vi "Make HTTP Request v4.vi"(5 "Request Options":T1={"request headers"=[], "request parameters"=[], "request body"="", "region handling"=enum."use region everywhere", "URL formatting"=enum."region."}, 7 "HTTP-Verb":string(combo)="GET", 8 "error in":errorcluster, 9 "URL Suffix":string, 10 "URL Prefix":string, 11 "AWS Core in":refnum<class "HTTP Request.lvclass">) -> (0 "error out":errorcluster, 1 "response body":string, 2 "response headers":string, 3 "AWS Core out":refnum<class "HTTP Request.lvclass">, 4 "Call Result":string)   [LabVIEW 2015, in "NI_AWS_Core.lvlib" / "HTTP Request.lvclass"]
uses:
  HTTP Request.lvclass
  Request Options.ctl
  Name Value Pair.ctl
  Region handling.ctl
  URL formatting.ctl
  HTTP Request.lvclass/HTTP Request.ctl
  Read Credentials.vi
  Read Service.vi
  Read Verify Server.vi
  <vilib>/httpClient/LabVIEWHTTPClient.lvlib
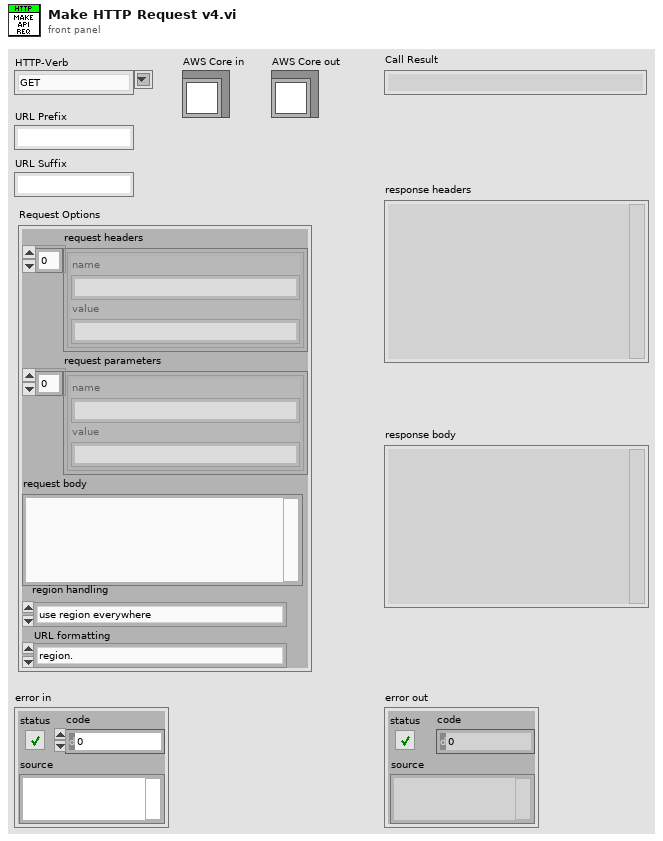
[diagram p1: front panel]
types:
  T1 = typedef "NI_AWS_Core.lvlib/HTTP Request.lvclass/Request Options.ctl" = cluster{"request headers":T2[], "request parameters":T2[], "request body":string, "region handling":T3, "URL formatting":T4}
  T2 = typedef "NI_AWS_Core.lvlib/HTTP Request.lvclass/Name Value Pair.ctl" = cluster{"name":string, "value":string}
  T3 = typedef "NI_AWS_Core.lvlib/HTTP Request.lvclass/Region handling.ctl" = enum16{"use region everywhere", "use region (authentication only)", "use region (URL only)", "ignore region everwhere"}
  T4 = typedef "NI_AWS_Core.lvlib/HTTP Request.lvclass/URL formatting.ctl" = enum16{"region-", "region."}
  T5 = typedef "AWS Core.lvlib/AWS Credentials.ctl" = cluster{"Access Key":string, "Secret Key":string}
  T6 = typedef "NI_AWS_Core.lvlib/HTTP Request.lvclass/Region.ctl" = enum16{"us-east-1", "us-east-2", "us-west-1", "us-west-2", "ap-northeast-1", "ap-northeast-2", "ap-southeast-1", "ap-southeast-2", "ca-central-1", "eu-central-1", "eu-west-1", "eu-west-2", "sa-east-1"}
  T7 = typedef "LabVIEWHTTPClient.lvlib/ClientHandle.ctl" = refnum<k1>
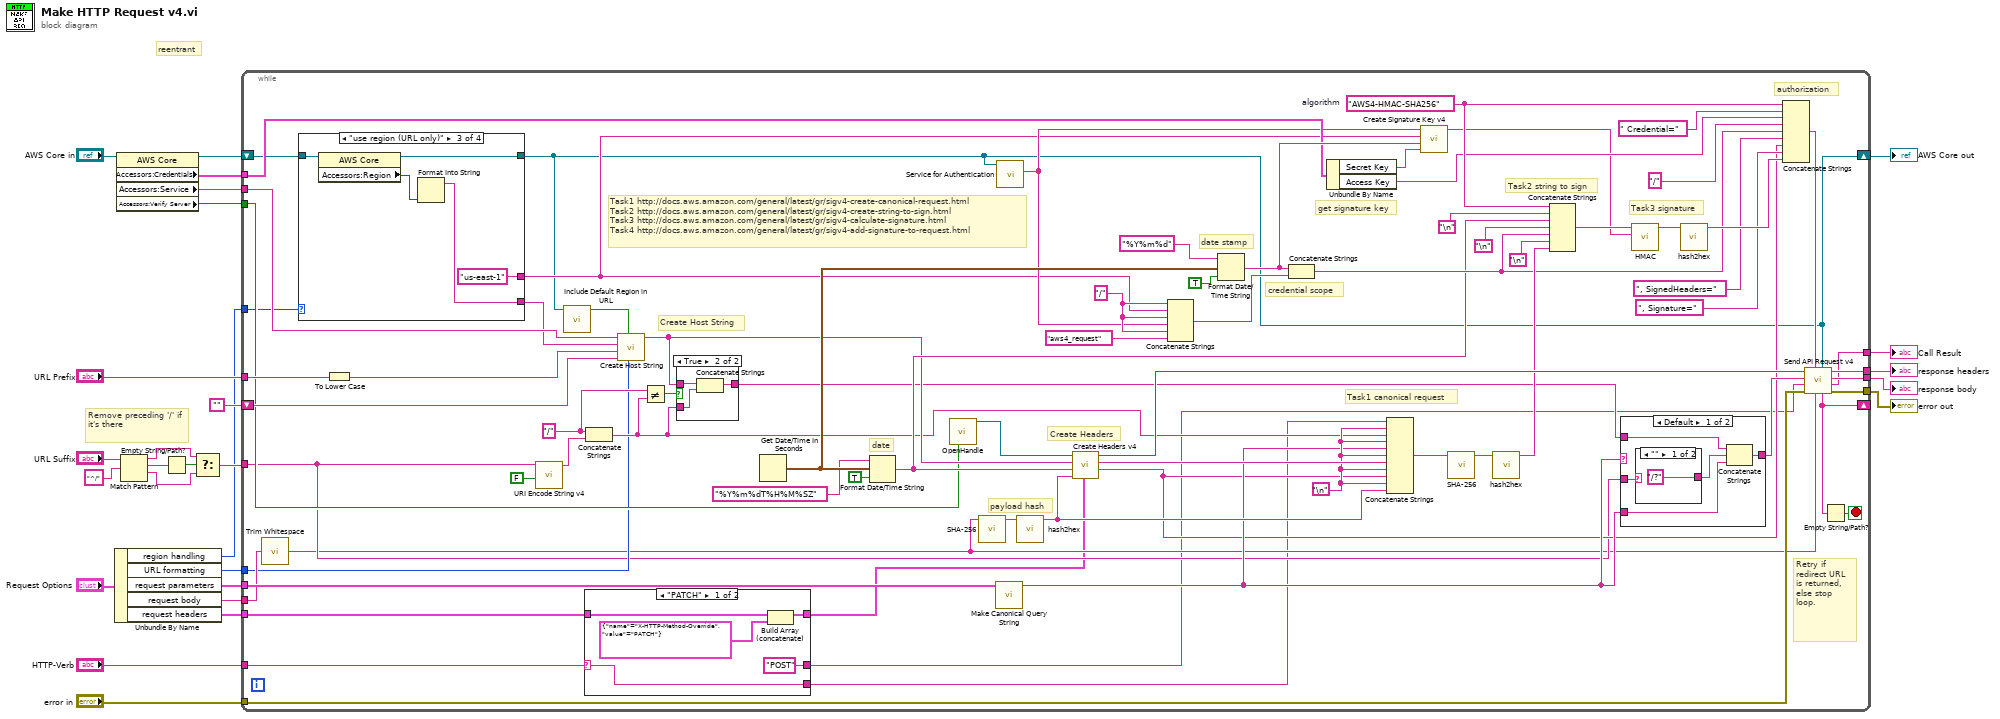
[diagram p0: block diagram]
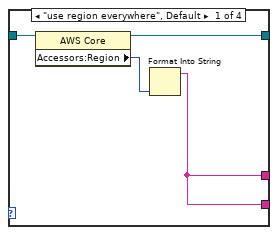
[diagram p3: hidden frame]
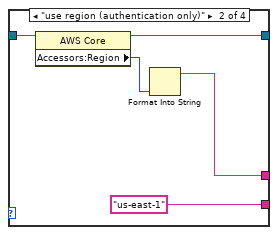
[diagram p4: hidden frame]
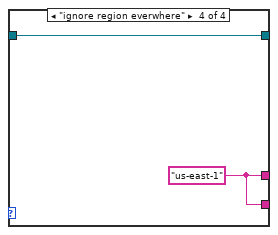
[diagram p5: hidden frame]
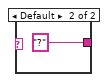
[diagram p7: hidden frame]
diagram:
  # "reentrant"
  # "Remove preceding '/' if it's there"
  n1 = Unbundle By Name("Request Options") -> ("region handling"=w3:T3, "URL formatting"=w2:T4, "request parameters"=w5:T2[], "request body"=w6:string, "request headers"=w4:T2[])
  n2 = property class="AWS Core"(reference="AWS Core in") -> (reference out=w11:refnum<class "HTTP Request.lvclass">, "Accessors:Credentials"=w10:T5, "Accessors:Service"=w9:string, "Accessors:Verify Server"=w8:bool)  [unwired: 1 in, 1 out]
  n3 = Match Pattern(string="URL Suffix", regular expression="^/") -> (before substring=w21:string, match substring=w19:string, after substring=w22:string)  [unwired: 1 in, 1 out]
  n4 = Empty String/Path?(string/path=w19) -> (empty?=w20:bool)
  n5 = Select(t=w21, s=w20, f=w22) -> (s? t:f=w17:string)
  n6 = while {
    tunnel: [w102] -> w27
    tunnel: [w55] -> w25
    tunnel: [w60] -> w24
    shift-right: [w59] -> _
    shift-left: "" ("Redirect endpoint") -> [w57]
    tunnel: [w56] -> w26
    tunnel: "error in" -> [w52]
    tunnel: w17 -> [w37]
    tunnel: "URL Prefix" -> [w48]
    tunnel: w5 -> [w47]
    tunnel: w6 -> [w46]
    tunnel: w4 -> [w34]
    tunnel: "HTTP-Verb" -> [w35]
    tunnel: w10 -> [w45]
    tunnel: w9 -> [w43]
    tunnel: w8 -> [w44]
    tunnel: w3 -> [w42]
    tunnel: w2 -> [w40]
    shift-right: [w29] -> w1
    shift-left: w11 -> [w39]
    stop <- w58 stop-if-true
    w65 = "/" ("string")
    w76 = "/" ("string")
    w94 = "AWS4-HMAC-SHA256"  # algorithm
    w72 = "\n"
    # "Retry if redirect URL is returned, else stop loop."
    # "Create Host String"
    # "Task1 canonical request"
    # "Create Headers"
    # "get signature key"
    # "Task1 http://docs.aws.amazon.com/general/latest/gr/sigv4-create-canonical-request.html\nTask2 http://docs.aws.amazon.com/general/latest/gr/sigv4-create-string-to-sign.html\nTask3 http://docs.aws.amazon.com/general/latest/gr/sigv4-calculate-signature.html\nTask4 http://docs.aws.amazon.com/general/latest/gr/sigv4-add-signature-to-request.html"
    # "date stamp"
    # "date"
    # "payload hash"
    # "authorization"
    # "Task3 signature"
    # "Task2 string to sign"
    # "credential scope"
    n7 = call <vilib>:"Trim Whitespace.vi"("string"=w46) -> ("trimmed string"=w36:string)  [unwired: 1 in]
    n8 = case shown="\"use region (URL only)\"" w42 {
      tunnel: [w110 w114 "us-east-1" ("x") w125] -> w30
      tunnel: [w110 "us-east-1" ("x") w119 w125] -> w41
      tunnel: w39 -> [w112 w116 w121 w124]
      tunnel: [w111 w115 w120 w124] -> w29
      frame "use region everywhere", Default {
        n9 = property class="AWS Core"(reference=w112) -> (reference out=w111:refnum<class "HTTP Request.lvclass">, "Accessors:Region"=w113:T6)  [unwired: 1 in, 1 out]
        n10 = Format Into String(w113) -> (resulting string=w110:string)  [unwired: 3 in, 1 out]
      }
      frame "use region (authentication only)" {
        n11 = property class="AWS Core"(reference=w116) -> (reference out=w115:refnum<class "HTTP Request.lvclass">, "Accessors:Region"=w117:T6)  [unwired: 1 in, 1 out]
        n12 = Format Into String(w117) -> (resulting string=w114:string)  [unwired: 3 in, 1 out]
      }
      frame "use region (URL only)" {
        n13 = property class="AWS Core"(reference=w121) -> (reference out=w120:refnum<class "HTTP Request.lvclass">, "Accessors:Region"=w122:T6)  [unwired: 1 in, 1 out]
        n14 = Format Into String(w122) -> (resulting string=w119:string)  [unwired: 3 in, 1 out]
      }
      frame "ignore region everwhere" {
        w125 = "us-east-1" ("x")
      }
    }
    n15 = To Lower Case(string=w48) -> (all lower case string=w53:string)
    n16 = call "URI Encode String v4.vi"("Encode /"=FALSE, "Un-encoded String"=w37) -> ("UriEncoded String"=w50:string)  [unwired: 9 in]
    n17 = call-dynamic "Include Default Region in URL.vi"("AWS Core"=w29) -> ("Include Default Region"=w28:bool)  [unwired: 10 in]
    n18 = case shown="\"PATCH\"" w35 {
      selector: w35 -> [w104 w108]
      tunnel: w34 -> [w107 w109]
      tunnel: [w106 w109] -> w33
      tunnel: ["POST" w108] -> w32
      tunnel: [w104 w108] -> w31
      frame "PATCH" {
        n19 = Build Array (concatenate)(w107, T2 {"name"="X-HTTP-Method-Override", "value"="PATCH"} ("Cluster")) -> (w106:T2[])
      }
      frame Default {
      }
    }
    n20 = Concatenate Strings(w65, w50) -> (w62:string)
    n21 = call "Create Host String.vi"("URL formatting"=w40, "Include Default Region"=w28, "Redirect Endpoint"=w57, "URL Prefix"=w53, "Region"=w41, "AWS Service"=w43) -> ("Host String"=w63:string)  [unwired: 5 in]
    n22 = Not Equal?(x=w65, y=w62) -> (x != y?=w64:bool)
    n23 = case shown="True" w64 {
      tunnel: w63 -> [w126 w129]
      tunnel: w62 -> [_ w128]
      tunnel: [w126 w127] -> w61
      frame False {
      }
      frame True {
        n24 = Concatenate Strings(w129, w128) -> (w127:string)
      }
    }
    n25 = Get Date/Time In Seconds() -> (seconds since 1Jan1904=w69:timestamp)
    n26 = Format Date/Time String(time format string (%c)="%Y%m%dT%H%M%SZ", seconds (now)=w69, UTC format=TRUE) -> (date/time string=w70:string)
    n27 = call <vilib>:"OpenHandle.vi"("verify server(true)"=w44) -> ("client handle out"=w73:T7)  [unwired: 13 in, 1 out]
    n28 = call "SHA-256.vi"("Message"=w36) -> ("Hash Value"=w86:string)  [unwired: 10 in]
    n29 = call "Make Canonical Query String.vi"("request parameters"=w47) -> ("canonical parameters"=w66:string)  [unwired: 10 in]
    n30 = call-dynamic "Service for Authentication.vi"("HTTP Request"=w29) -> ("Service for Authentication"=w38:string)  [unwired: 10 in]
    n31 = call "hash2hex.vi"("hash string"=w86) -> ("hex string"=w71:string)  [unwired: 10 in]
    n32 = call "Create Headers v4.vi"("request headers"=w33, "RequestBody Payload"=w71, "date/time string"=w70, "Host"=w63, "Client Handle In"=w73) -> ("Signed Headers"=w54:string, "canonical headers"=w90:string, "Client Handle Out"=w100:T7)  [unwired: 3 in]
    n33 = Concatenate Strings(w76, w30, w76, w38, w76, "aws4_request" ("string")) -> (w77:string)
    n34 = Format Date/Time String(time format string (%c)="%Y%m%d", seconds (now)=w69, UTC format=TRUE) -> (date/time string=w83:string)
    n35 = Concatenate Strings(w83, w77) -> (w78:string)
    n36 = Unbundle By Name(w45) -> ("Secret Key"=w74:string, "Access Key"=w80:string)
    n37 = Concatenate Strings(w31, w72, w62, w72, w66, w72, w90, w72, w54, w72, w71) -> (w85:string)
    n38 = call "Create Signature Key v4.vi"("AWS Service"=w38, "Region"=w30, "date/time string"=w83, "Secret Key"=w74) -> ("Keyed-Hash"=w51:string)  [unwired: 6 in]
    n39 = call "SHA-256.vi"("Message"=w85) -> ("Hash Value"=w84:string)  [unwired: 10 in]
    n40 = call "hash2hex.vi"("hash string"=w84) -> ("hex string"=w93:string)  [unwired: 10 in]
    n41 = Concatenate Strings(w94, "\n", w70, "\n", w78, "\n", w93) -> (w82:string)
    n42 = case shown="Default" w66 {
      tunnel: [w134 w137] -> w67
      tunnel: w61 -> [w132 w137]
      tunnel: w66 -> [w133 _]
      tunnel: w37 -> [w130 _]
      frame Default {
        n43 = case shown="\"\"" w130 {
          tunnel: ["/?" ("string") "?" ("string")] -> w131
          frame "" {
          }
          frame Default {
          }
        }
        n44 = Concatenate Strings(w132, w131, w133) -> (w134:string)
      }
      frame "" {
      }
    }
    n45 = call "HMAC.vi"("Key"=w51, "Message"=w82) -> ("Keyed Hash"=w81:string)  [unwired: 9 in]
    n46 = call "hash2hex.vi"("hash string"=w81) -> ("hex string"=w99:string)  [unwired: 10 in]
    n47 = Concatenate Strings(w94, " Credential=", w80, "/", w78, ", SignedHeaders=", w54, ", Signature=", w99) -> (w101:string)
    n48 = call "Send API Request v4.vi"("AWS Core"=w29, "request body"=w36, "Authorization"=w101, "error in (no error)"=w52, "HTTP-Verb"=w32, "Host String"=w67, "Client Handle"=w100) -> ("error out"=w55:errorcluster, "Call Result"=w56:string, "response body"=w60:string, "response headers"=w102:string, "Redirect endpoint"=w59:string)
    n49 = Empty String/Path?(string/path=w59) -> (empty?=w58:bool)
  }
  "response headers" <- w27
  "response body" <- w24
  "error out" <- w25
  "Call Result" <- w26
  "AWS Core out" <- w1
